vi "ABGates.vi"(9 "N":dbl=2.0, 11 "# of loop":i32) -> (0 "B Gate":dbl[](array[numeric]), 1 "A Gate":dbl[](array[numeric]), 2 "average A-B/A+B":dbl)   [LabVIEW 2024]
uses:
  Global_Stop.vi
panel:
  out "A-B/A+B":dbl[](array[numeric])
  in  "Number of passes A and B to give final value":i32=25
  out "Waveform Chart":dbl(graph)
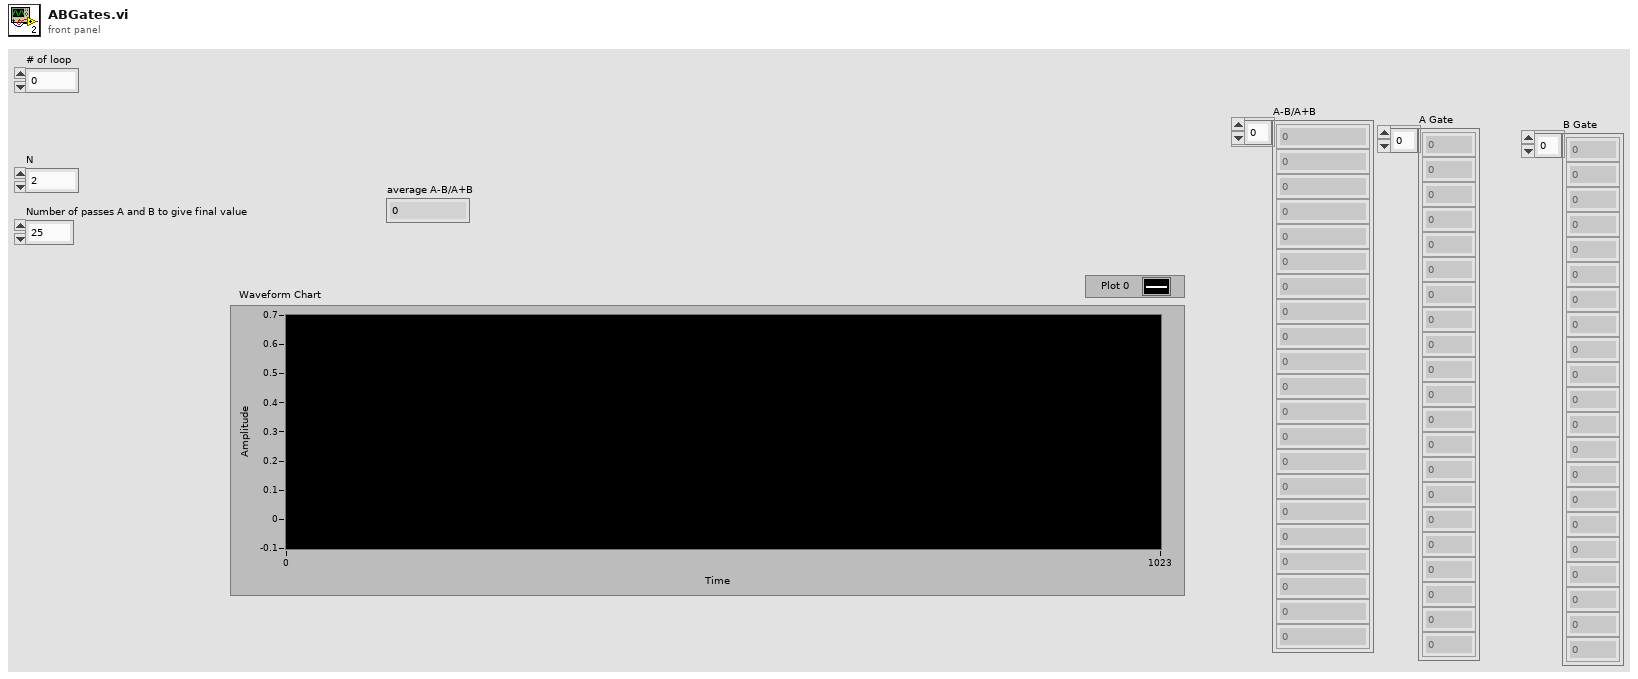
[diagram p1: front panel]
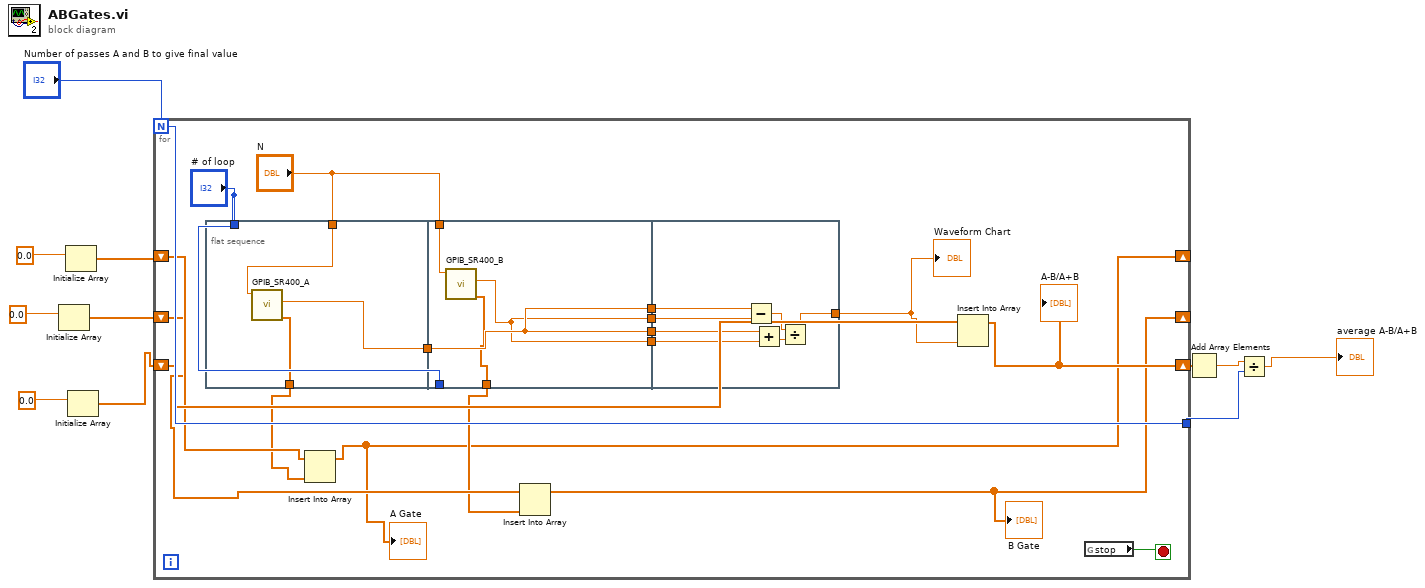
[diagram p0: block diagram]
diagram:
  n1 = Initialize Array "Initialize Array"(0.0 ("element")) -> (w2:dbl[])  [unwired: 1 in]
  n2 = Initialize Array "Initialize Array"(0.0 ("element")) -> (w1:dbl[])  [unwired: 1 in]
  n3 = Initialize Array "Initialize Array"(0.0 ("element")) -> (w9:dbl[])  [unwired: 1 in]
  n4 = for {
    N: "Number of passes A and B to give final value" -> [w23]
    shift-right: [w21] -> w8
    shift-left: w9 -> [w22]
    tunnel: [w23] -> w6
    shift-right: [w14] -> _
    shift-left: w2 -> [w16]
    shift-right: [w13] -> _
    shift-left: w1 -> [w18]
    stop <- w12 stop-if-true
    n5 = flat-sequence {
      tunnel: [w31] -> w29
      tunnel: "N" -> [w32]
      tunnel: "# of loop" -> [_]
      tunnel: [w30] -> w17
      tunnel: [w36] -> w28
      tunnel: w29 -> [w36]
      tunnel: [w34] -> w27
      tunnel: [w36] -> w26
      tunnel: [w34] -> w25
      tunnel: "N" -> [w35]
      tunnel: "# of loop" -> [_]
      tunnel: [w33] -> w15
      tunnel: [w37] -> w20
      tunnel: w28 -> [w43]
      tunnel: w27 -> [w42]
      tunnel: w26 -> [w41]
      tunnel: w25 -> [w40]
      frame #0 {
        n6 = call "GPIB_SR400_A.vi"("N per point"=w32) -> ("A Gate"=w30:dbl[], "x/y"=w31:dbl)  [unwired: 9 in]
      }
      frame #1 {
        n7 = call "GPIB_SR400_B.vi"("N per point"=w35) -> ("B Gate"=w33:dbl[], "x/y"=w34:dbl)  [unwired: 9 in]
      }
      frame #2 {
        n8 = Subtract(x=w43, y=w42) -> (x-y=w39:dbl)
        n9 = Add(x=w41, y=w40) -> (x+y=w38:dbl)
        n10 = Divide(x=w39, y=w38) -> (x/y=w37:dbl)
      }
    }
    n11 = Insert Into Array(array=w18, new element=w17) -> (w13:dbl[])  [unwired: 1 in]
    "A Gate" <- w13
    n12 = Insert Into Array(array=w16, new element=w15) -> (w14:dbl[])  [unwired: 1 in]
    "B Gate" <- w14
    n13 = Insert Into Array(array=w22, new element=w20) -> (w21:dbl[])  [unwired: 1 in]
    "A-B/A+B" <- w21
    n14 = global read "Global_Stop.vi" "stop"() -> (w12:bool)
    "Waveform Chart" <- w20
  }
  n15 = Add Array Elements(numeric array=w8) -> (sum=w7:dbl)
  n16 = Divide(x=w7, y=w6) -> (x/y=→"average A-B/A+B":dbl)
